vi "PositionCtrl_DriveFwdBck_Example.vi"() -> ()   [LabVIEW 2019]
uses:
  <vilib>/Rock Robotics/WPI/ThirdParty/JAS_Junk/TrajLib/Util_GetTime.vi
  <vilib>/Rock Robotics/WPI/ThirdParty/JAS_Junk/TrajLib/VI/MathUtil_RateOfChange.vi
  <vilib>/Rock Robotics/WPI/ThirdParty/JAS_Junk/TrajLib/SlewRateLimiter_New.vi
  <vilib>/Rock Robotics/WPI/ThirdParty/JAS_Junk/TrajLib/SlewRateLimiter_Reset.vi
  <vilib>/Rock Robotics/WPI/ThirdParty/JAS_Junk/TrajLib/SlewRateLimiter_Calculate.vi
  <vilib>/Rock Robotics/WPI/ThirdParty/JAS_Junk/TrajLib/SlewRateLimiter_SetRate.vi
  <vilib>/Rock Robotics/WPI/ThirdParty/JAS_Junk/TrajLib/VI/Util_GetTime_U32.vi
  <vilib>/Rock Robotics/WPI/ThirdParty/JAS_Junk/TrajLib/VI/Util_GetTime_U64.vi
  <vilib>/Rock Robotics/WPI/ThirdParty/JAS_Junk/TrajLib/Trajectory_Library.lvlib
panel:
  out "Targets along the way":cluster{dbl, "PositionError":dbl, dbl}(graph)
  in  "SP - Desired Position\n (Inch)":dbl(slide) scale=-10.0..350.0
  out "PV - Current Position\n (Inch)":dbl(slide) scale=-10.0..350.0
  out "Goal":T1(graph)
  out "Motor Output":dbl format="%13.3f"
  out "AtGoal":bool
  out "PositionError  \n(Inch)":dbl format="%13.2f"
  out "Velocity  (Inch/Sec)":dbl format="%13.2f"
  out "Velocity  \n(Inch/Sec) 2":dbl format="%13.2f"
  out "Kp":dbl format="%#_13g"
  in  "Position\nDeadband (Inch)":dbl=0.08 format="%#_13g"
  in  "Output Deadband\n(mot units)":dbl=0.08 format="%#_13g"
  in  "Kd":dbl format="%#_13g"
  in  "Position Threshold\n(inch)":dbl=50.0 format="%#_13g"
  # "Position has hard limit\n at -5 and 300 inches"
  # "BASIC TUNING"
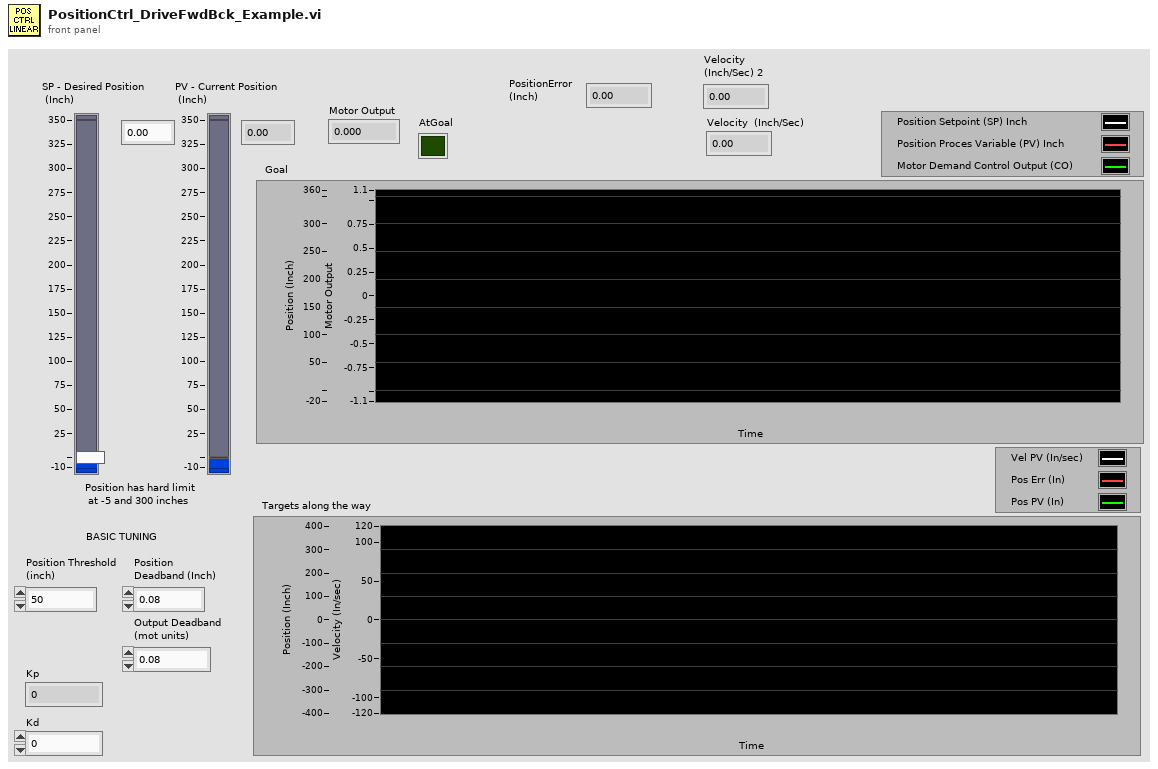
[diagram p1: front panel]
types:
  T1 = cluster{"SP - Desired Position\n (Inch)":dbl, "upper limit":dbl, "upper limit":dbl}
  T2 = typedef "Trajectory_Library.lvlib/PosCtrl_Tuning_Type.ctl" = cluster{"Slope":dbl, "Offset":dbl, "Error Deadband":dbl, "At Reference Count":i32, "Negate Output":bool, "Max Allowd Position":dbl, "Min Allowd Position":dbl, "Kd":dbl}
  T3 = cluster{"SP - Desired Position\n (Inch)":dbl, dbl, "Output":dbl}
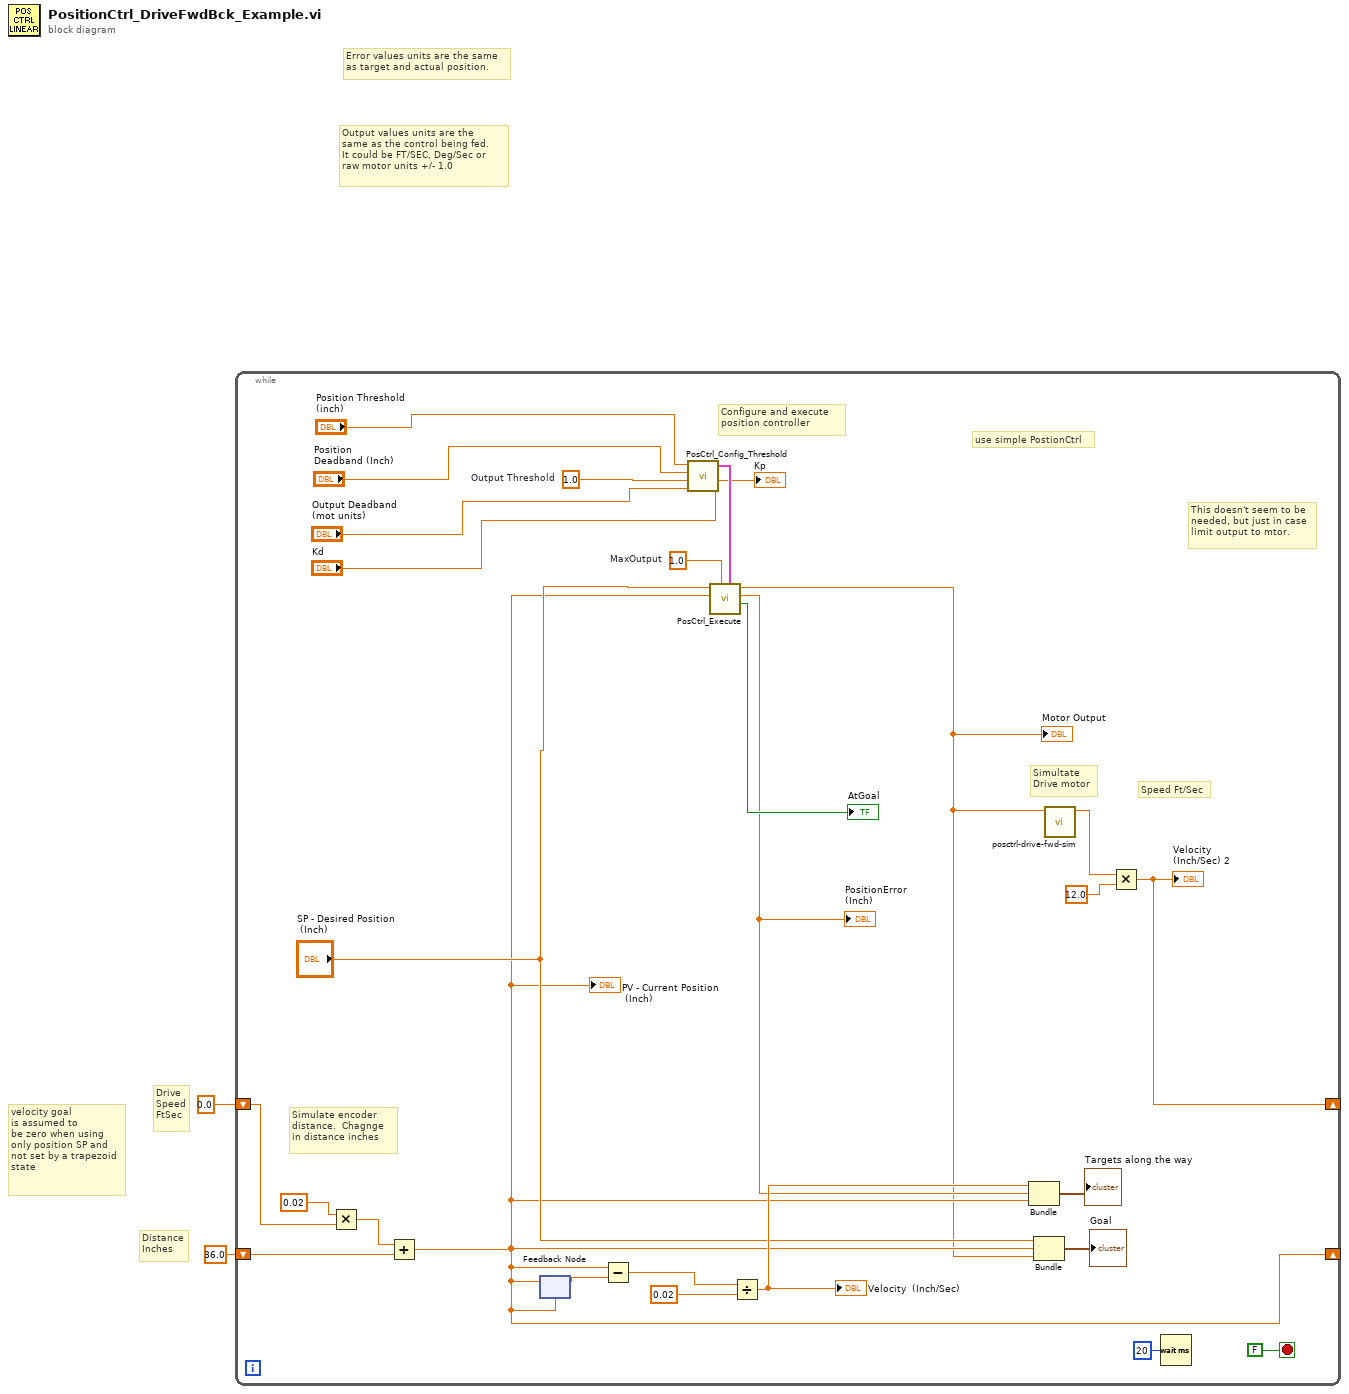
[diagram p0: block diagram]
diagram:
  # "Output values units are the\nsame as the control being fed.  \nIt could be FT/SEC, Deg/Sec or\nraw motor units +/- 1.0"
  # "Error values units are the same \nas target and actual position."
  # "velocity goal\nis assumed to \nbe zero when using\nonly position SP and\nnot set by a trapezoid\nstate"
  # "Distance\nInches"
  # "Drive\nSpeed\nFtSec"
  n1 = while {
    shift-right: [w11] -> _
    shift-left: 36.0 ("upper limit") -> [w22]
    shift-right: [w16] -> _
    shift-left: 0.0 ("upper limit") -> [w19]
    stop <- FALSE stop-if-true
    w14 = 1.0  # MaxOutput
    w13 = 1.0  # Output Threshold
    # "Configure and execute \nposition controller"
    # "This doesn't seem to be\nneeded, but just in case\nlimit output to mtor."
    # "use simple PostionCtrl"
    # "Speed Ft/Sec"
    # "Simultate \nDrive motor"
    # "Simulate encoder \ndistance.  Chagnge \nin distance inches"
    n2 = Multiply(x=0.02 ("value"), y=w19) -> (x*y=w24:dbl)
    n3 = Add(x=w24, y=w22) -> (x+y=w11:dbl)
    "PV - Current Position\n (Inch)" <- w11
    n4 = feedback-in #1(w11) -> ()
    n5 = feedback #1(w11) -> (w28:dbl)
    n6 = Subtract(x=w11, y=w28) -> (x-y=w27:dbl)
    n7 = call <vilib>:"PosCtrl_Config_Threshold.vi"("Kd"="Kd", "Output Deadband"="Output Deadband\n(mot units)", "Output Threshold"=w13, "ErrorDeadband"="Position\nDeadband (Inch)", "ErrorThreshold"="Position Threshold\n(inch)") -> ("Kp"=→"Kp":dbl, "PosCtrl_Config_Params"=w15:T2)  [unwired: 5 in]
    n8 = call <vilib>:"PosCtrl_Execute.vi"("PosCtrl_Config_Params"=w15, "MaxOutput"=w14, "CurrentPosition"=w11, "TargetPosition"="SP - Desired Position\n (Inch)") -> ("OnTarget"=→"AtGoal":bool, "PositionError"=w6:dbl, "Output"=w3:dbl)  [unwired: 5 in]
    "Motor Output" <- w3
    "PositionError  \n(Inch)" <- w6
    n9 = Divide(x=w27, y=0.02) -> (x/y=w20:dbl)
    "Velocity  (Inch/Sec)" <- w20
    n10 = Bundle(w20, "PositionError"=w6, w11) -> (→"Targets along the way":cluster{dbl, "PositionError":dbl, dbl})  [unwired: 1 in]
    n11 = Bundle("SP - Desired Position\n (Inch)"="SP - Desired Position\n (Inch)", w11, "Output"=w3) -> (→"Goal":T3)  [unwired: 1 in]
    n12 = call "posctrl-drive-fwd-sim.vi"("Motor Demand"=w3) -> ("Drive Speed Ft/Sec"=w18:dbl)  [unwired: 10 in]
    n13 = Multiply(x=w18, y=12.0) -> (x*y=w16:dbl)
    "Velocity  \n(Inch/Sec) 2" <- w16
    n14 = Wait (ms)(milliseconds to wait=u32 20) -> ()  [unwired: 1 out]
  }
